vi "Dialog Box.vi"(8 "error in (no error)":errorcluster, 11 "Dialog in":refnum<class "Dialog.lvclass">) -> (0 "error out":errorcluster, 1 "timed out?":bool, 2 "Selection":string, 3 "Dialog out":refnum<class "Dialog.lvclass">)   [LabVIEW 2012, in "Dialog.lvlib" / "Dialog.lvclass"]
doc: "This VI contains the code for the dialog box.\nOverride this VI to provide more functionality or to create your own application-specific dialog box."
uses:
  Dialog.lvclass
  Fading/_Fade In(I32).vi
panel:
  out "String":string
  in  "OK Button":bool
  # "Message"
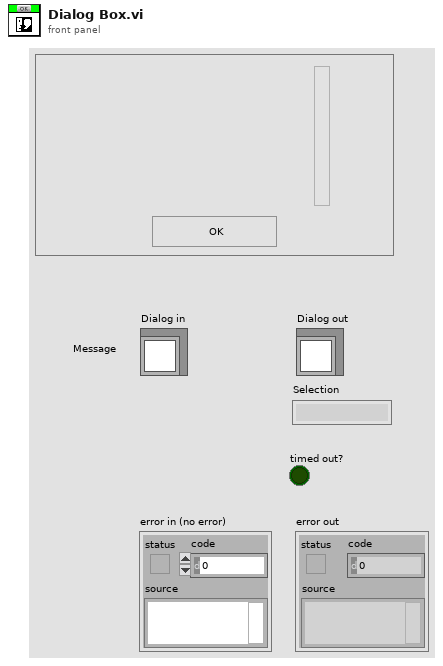
[diagram p1: front panel]
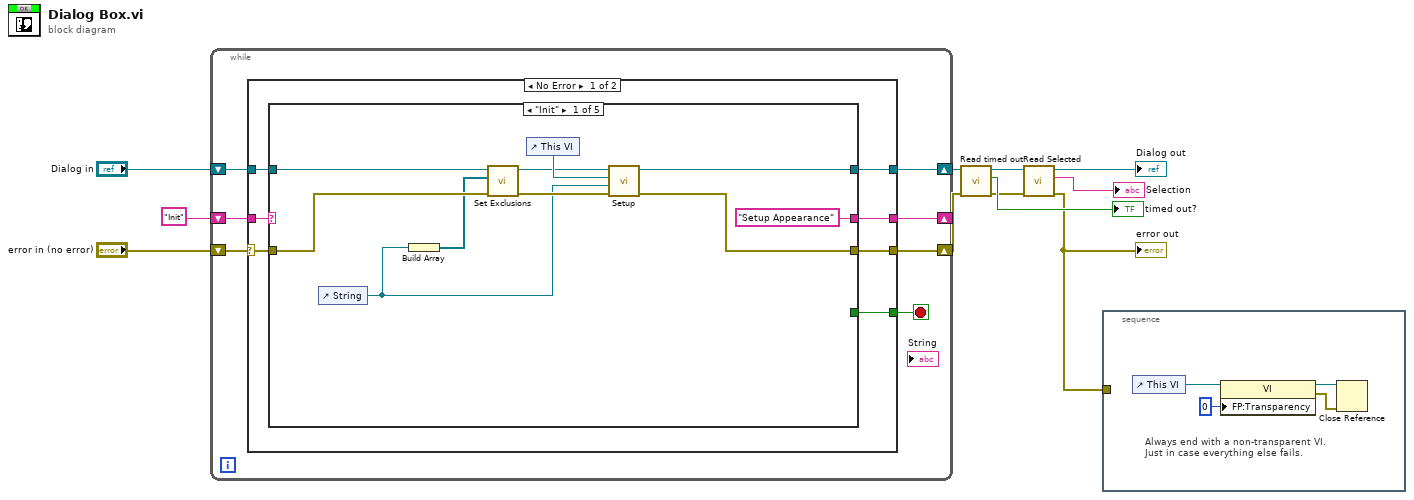
[diagram p0: block diagram]
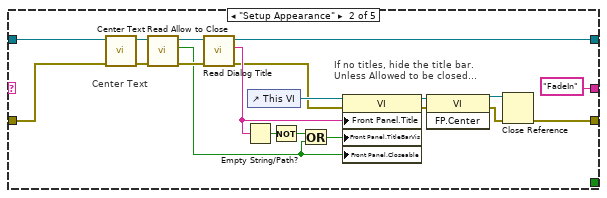
[diagram p2: hidden frame]
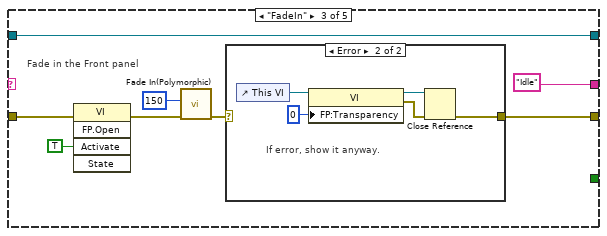
[diagram p3: hidden frame]
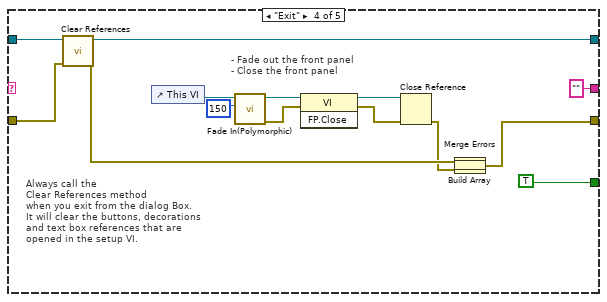
[diagram p5: hidden frame]
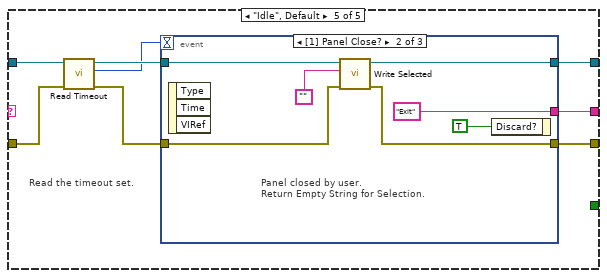
[diagram p6: hidden frame]
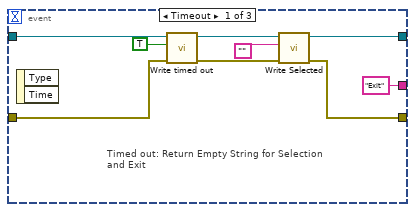
[diagram p7: hidden frame]
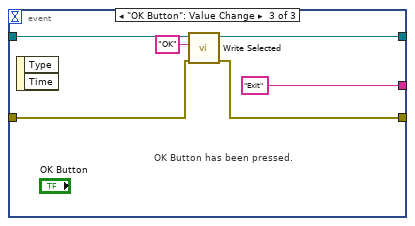
[diagram p8: hidden frame]
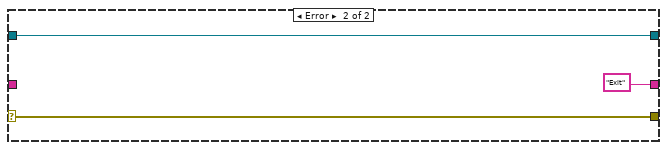
[diagram p9: hidden frame]
diagram:
  n1 = while {
    shift-right: [w14] -> _
    shift-left: "Init" -> [w15]
    shift-right: [w18] -> w4
    shift-left: "Dialog in" -> [w17]
    shift-right: [w16] -> w3
    shift-left: "error in (no error)" -> [w12]
    stop <- w13 stop-if-true
    n2 = case shown="No Error" w12 {
      selector: w12 -> [w19 w117]
      tunnel: [w25 w115] -> w18
      tunnel: w17 -> [w24 w115]
      tunnel: [w23 w117] -> w16
      tunnel: w15 -> [w22 _]
      tunnel: [w21 "Exit"] -> w14
      tunnel: [w20 _] -> w13
      frame No Error {
        n3 = case shown="\"Init\"" w22 {
          tunnel: [w33 w46 w63 w79 w92] -> w25
          tunnel: w24 -> [w32 w37 w63 w80 w89]
          tunnel: [w26 w47 w59 w75 w91] -> w23
          tunnel: w19 -> [w29 w36 w58 w78 w86]
          tunnel: ["Setup Appearance" "FadeIn" "Idle" "" w90] -> w21
          tunnel: [_ _ _ TRUE _] -> w20
          frame "Init" {
            n4 = control-ref of="String"() -> (w28:refnum<vi>)
            n5 = Build Array(w28) -> (w27:refnum<vi>[])
            n6 = call-dynamic "Set Exclusions.vi"("error in (no error)"=w29, "Exclusions"=w27, "Dialog in"=w32) -> ("error out"=w30:errorcluster, "Dialog out"=w31:refnum<class "Dialog.lvclass">)  [unwired: 7 out]
            n7 = control-ref of="This VI"() -> (w34:refnum<vi>)
            n8 = call-dynamic "Setup.vi"("error in (no error)"=w30, "Str Refnum"=w28, "VI Reference"=w34, "Dialog in"=w31) -> ("error out"=w26:errorcluster, "Dialog out"=w33:refnum<class "Dialog.lvclass">)  [unwired: 6 out]
          }
          frame "Setup Appearance" {
            # "Center Text"
            # "If no titles, hide the title bar.\nUnless Allowed to be closed..."
            n9 = call-dynamic "Center Text.vi"("error in (no error)"=w36, "Dialog in"=w37) -> ("error out"=w42:errorcluster, "Dialog out"=w44:refnum<class "Dialog.lvclass">)  [unwired: 1 in, 7 out]
            n10 = call-dynamic "Read Allow to Close.vi"("error in (no error)"=w42, "Dialog.lvclass in"=w44) -> ("error out"=w41:errorcluster, "Allow to close?"=w38:bool, "Dialog.lvclass out"=w43:refnum<class "Dialog.lvclass">)  [unwired: 7 out]
            n11 = call-dynamic "Read Dialog Title.vi"("error in (no error)"=w41, "Dialog in"=w43) -> ("error out"=w45:errorcluster, "Dialog Title"=w50:string, "Dialog out"=w46:refnum<class "Dialog.lvclass">)  [unwired: 7 out]
            n12 = Empty String/Path?(string/path=w50) -> (empty?=w53:bool)
            n13 = control-ref of="This VI"() -> (w54:refnum<vi>)
            n14 = Not(x=w53) -> (.not. x?=w40:bool)
            n15 = Or(x=w40, y=w38) -> (x .or. y?=w39:bool)
            n16 = property class="VI"(reference=w54, error in=w45, "Front Panel.Title"=w50, "Front Panel.TitleBarVis"=w39, "Front Panel.Closeable"=w38) -> (reference out=w52:refnum<vi>, error out=w51:errorcluster)
            n17 = invoke class="VI" method="FP.Center"(reference=w52, error in=w51) -> (reference out=w49:refnum<vi>, error out=w48:errorcluster)  [unwired: 1 in, 1 out]
            n18 = Close Reference(reference=w49, error in (no error)=w48) -> (error out=w47:errorcluster)
          }
          frame "FadeIn" {
            # "Fade in the Front panel"
            n19 = invoke class="VI" method="FP.Open"(error in=w58, "Activate"=TRUE ("Front Panel Window:Open")) -> (error out=w57:errorcluster)  [unwired: 3 in, 4 out]
            n20 = call-poly "Fade In(Polymorphic).vi"("error in"=w57, "Fade time (ms)"=150) -> ("error out"=w60:errorcluster)  [unwired: 2 in, 7 out]
            n21 = case shown="Error" w60 {
              selector: w60 -> [w64 _]
              tunnel: [w64 w65] -> w59
              frame No Error {
              }
              frame Error {
                # "If error, show it anyway."
                n22 = control-ref of="This VI"() -> (w67:refnum<vi>)
                n23 = property class="VI"(reference=w67, "FP:Transparency"=u8 0 ("Front Panel Window:Transparency")) -> (reference out=w68:refnum<vi>, error out=w69:errorcluster)  [unwired: 1 in]
                n24 = Close Reference(reference=w68, error in (no error)=w69) -> (error out=w65:errorcluster)
              }
            }
          }
          frame "Exit" {
            # "Always call the\nClear References method\nwhen you exit from the dialog Box.\nIt will clear the buttons, decorations\nand text box references that are \nopened in the setup VI."
            # "- Fade out the front panel\n- Close the front panel"
            n25 = call-dynamic "Clear References.vi"("error in (no error)"=w78, "Dialog in"=w80) -> ("error out"=w77:errorcluster, "Dialog out"=w79:refnum<class "Dialog.lvclass">)  [unwired: 8 out]
            n26 = control-ref of="This VI"() -> (w81:refnum<vi>)
            n27 = call-poly "Fade In(Polymorphic).vi"("Fade time (ms)"=150, "VI Reference (calling VI)"=w81) -> ("error out"=w72:errorcluster, "dup VI Reference"=w73:refnum<vi>)  [unwired: 2 in, 6 out]
            n28 = invoke class="VI" method="FP.Close"(reference=w73, error in=w72) -> (reference out=w71:refnum<vi>, error out=w70:errorcluster)  [unwired: 1 in, 1 out]
            n29 = Close Reference(reference=w71, error in (no error)=w70) -> (error out=w76:errorcluster)
            n30 = Build Array(w77, w76) -> (w74:errorcluster[])
            n31 = Merge Errors(w74) -> (w75:errorcluster)
          }
          frame "Idle", Default {
            # "Read the timeout set."
            n32 = call-dynamic "Read Timeout.vi"("error in (no error)"=w86, "Dialog.lvclass in"=w89) -> ("error out"=w85:errorcluster, "Timeout"=w87:i32, "Dialog.lvclass out"=w88:refnum<class "Dialog.lvclass">)  [unwired: 7 out]
            n33 = event shown="[1] Panel Close?" {
              selector: _ -> [_ _ _]
              dyn-events: _ -> [_ _ _]
              timeout: w87 -> [_ _ _]
              tunnel: [w94 w104 w112] -> w92
              tunnel: w88 -> [w100 w105 w113]
              tunnel: [w95 w102 w109] -> w91
              tunnel: w85 -> [w98 w103 w110]
              tunnel: ["Exit" "Exit" "Exit"] -> w90
              event Timeout {
                # "Timed out: Return Empty String for Selection\nand Exit"
                n34 = event-data() -> ()  [unwired: 3 out]
                n35 = call-dynamic "Write timed out.vi"("error in (no error)"=w98, "timed out?"=TRUE, "Dialog.lvclass in"=w100) -> ("error out"=w96:errorcluster, "Dialog.lvclass out"=w97:refnum<class "Dialog.lvclass">)  [unwired: 7 out]
                n36 = call-dynamic "Write Selected.vi"("error in (no error)"=w96, "Selected"="", "Dialog.lvclass in"=w97) -> ("error out"=w95:errorcluster, "Dialog.lvclass out"=w94:refnum<class "Dialog.lvclass">)  [unwired: 7 out]
              }
              event Panel Close? {
                # "Panel closed by user.\nReturn Empty String for Selection."
                n37 = event-data() -> ()  [unwired: 4 out]
                n38 = call-dynamic "Write Selected.vi"("error in (no error)"=w103, "Selected"="", "Dialog.lvclass in"=w105) -> ("error out"=w102:errorcluster, "Dialog.lvclass out"=w104:refnum<class "Dialog.lvclass">)  [unwired: 7 out]
                n39 = event-data("Discard?"=TRUE) -> ()  [unwired: 1 in, 1 out]
              }
              event "OK Button": Value Change {
                # "OK Button has been pressed."
                n40 = event-data() -> ()  [unwired: 3 out]
                n41 = call-dynamic "Write Selected.vi"("error in (no error)"=w110, "Selected"="OK", "Dialog.lvclass in"=w113) -> ("error out"=w109:errorcluster, "Dialog.lvclass out"=w112:refnum<class "Dialog.lvclass">)  [unwired: 7 out]
              }
            }
          }
        }
      }
      frame Error {
      }
    }
  }
  n42 = call-dynamic "Read timed out.vi"("error in (no error)"=w3, "Dialog.lvclass in"=w4) -> ("error out"=w1:errorcluster, "timed out?"=→"timed out?":bool, "Dialog.lvclass out"=w2:refnum<class "Dialog.lvclass">)  [unwired: 7 out]
  n43 = call-dynamic "Read Selected.vi"("error in (no error)"=w1, "Dialog.lvclass in"=w2) -> ("error out"=w6:errorcluster, "Selected"=→"Selection":string, "Dialog.lvclass out"=→"Dialog out":refnum<class "Dialog.lvclass">)  [unwired: 7 out]
  "error out" <- w6
  n44 = stacked-sequence {
    tunnel: w6 -> [_]
    frame #0 {
      # "Always end with a non-transparent VI.\nJust in case everything else fails."
      n45 = control-ref of="This VI"() -> (w120:refnum<vi>)
      n46 = property class="VI"(reference=w120, "FP:Transparency"=u8 0 ("Front Panel Window:Transparency")) -> (reference out=w119:refnum<vi>, error out=w118:errorcluster)  [unwired: 1 in]
      n47 = Close Reference(reference=w119, error in (no error)=w118) -> ()  [unwired: 1 out]
    }
  }
